vi "NV-ESR_Initialization.vi"() -> ()   [LabVIEW 2024]
panel:
  in  "Instructions":T1(array[cluster])=[{"Instruct Data"=0, "Op Code"=0, "Flags"=[FALSE, TRUE, TRUE, FALSE, FALSE, FALSE, FALSE, FALSE, FALSE, FALSE, FALSE, FALSE, FALSE, FALSE, FALSE, FALSE, FALSE, FALSE, FALSE, FALSE, FALSE, FALSE, FALSE, TRUE], "Comments"="0", "Time (s)"=1e-07}, {"Instruct Data"=0, "Op Code"=0, "Flags"=[TRUE, TRUE, FALSE, TRUE, FALSE, FALSE, FALSE, FALSE, FALSE, FALSE, FALSE, FALSE, FALSE, FALSE, FALSE, FALSE, FALSE, FALSE, FALSE, FALSE, FALSE, FALSE, FALSE, FALSE], "Comments"="1 MW", "Time (s)"=2e-06}, {"Instruct Data"=0, "Op Code"=6, "Flags"=[FALSE, TRUE, FALSE, FALSE, FALSE, FALSE, FALSE, FALSE, FALSE, FALSE, FALSE, FALSE, FALSE, FALSE, FALSE, FALSE, FALSE, FALSE, FALSE, FALSE, FALSE, FALSE, FALSE, FALSE], "Comments"="2 AOM delay", "Time (s)"=2e-06}, {"Instruct Data"=0, "Op Code"=0, "Flags"=[FALSE, TRUE, FALSE, FALSE, FALSE, FALSE, FALSE, FALSE, FALSE, FALSE, FALSE, FALSE, FALSE, FALSE, FALSE, FALSE, FALSE, FALSE, FALSE, FALSE, FALSE, FALSE, FALSE, FALSE], "Comments"="3 read", "Time (s)"=3e-07}, {"Instruct Data"=0, "Op Code"=0, "Flags"=[FALSE, TRUE, FALSE, FALSE, FALSE, FALSE, FALSE, TRUE, FALSE, FALSE, FALSE, FALSE, FALSE, FALSE, FALSE, FALSE, FALSE, FALSE, FALSE, FALSE, FALSE, FALSE, FALSE, FALSE], "Comments"="4 AOM", "Time (s)"=2.2e-06}, {"Instruct Data"=0, "Op Code"=6, "Flags"=[FALSE, FALSE, FALSE, FALSE, FALSE, FALSE, FALSE, TRUE, FALSE, FALSE, FALSE, FALSE, FALSE, FALSE, FALSE, FALSE, FALSE, FALSE, FALSE, FALSE, FALSE, FALSE, FALSE, FALSE], "Comments"="5", "Time (s)"=5e-06}, {"Instruct Data"=0, "Op Code"=6, "Flags"=[FALSE, TRUE, TRUE, FALSE, FALSE, FALSE, FALSE, FALSE, FALSE, FALSE, FALSE, FALSE, FALSE, FALSE, FALSE, FALSE, FALSE, FALSE, FALSE, FALSE, FALSE, FALSE, FALSE, FALSE], "Comments"="6", "Time (s)"=3e-06}, {"Instruct Data"=0, "Op Code"=0, "Flags"=[FALSE, TRUE, FALSE, FALSE, FALSE, FALSE, FALSE, FALSE, FALSE, FALSE, FALSE, FALSE, FALSE, FALSE, FALSE, FALSE, FALSE, FALSE, FALSE, FALSE, FALSE, FALSE, FALSE, FALSE], "Comments"="7", "Time (s)"=1e-06}, {"Instruct Data"=0, "Op Code"=0, "Flags"=[FALSE, TRUE, FALSE, FALSE, FALSE, FALSE, FALSE, FALSE, FALSE, FALSE, FALSE, FALSE, FALSE, FALSE, FALSE, FALSE, FALSE, FALSE, FALSE, FALSE, FALSE, FALSE, FALSE, FALSE], "Comments"="8", "Time (s)"=1e-06}, {"Instruct Data"=0, "Op Code"=0, "Flags"=[FALSE, TRUE, FALSE, FALSE, FALSE, FALSE, FALSE, FALSE, FALSE, FALSE, FALSE, FALSE, FALSE, FALSE, FALSE, FALSE, FALSE, FALSE, FALSE, FALSE, FALSE, FALSE, FALSE, FALSE], "Comments"="9", "Time (s)"=1e-06}] {"Time (s)" format="%.3p"; "Op Code" items=["Continue", "Stop", "Loop", "End Loop", "JSR", "RTS", "Branch", "Long Delay", "Wait"]}
  in  "Path to spinapi.dll":path=path "C:/SpinCore/SpinAPI/lib/spinapi64.dll"
  in  "# of Instructions":u32=3
  in  "clock_freq (MHz)":dbl=500.0
  # "1) MW indication\n2)AOM\n3) SR400 Trigger\n4)I\n5)Q\n24) Scope Trigger"
  # "1"
  # "2"
  # "3"
  # "4"
  # "5"
  # "6"
  # "7"
  # "8"
  # "9"
  # "10"
  # "11"
  # "12"
  # "13"
  # "14"
  # "15"
  # "16"
  # "17"
  # "18"
  # "19"
  # "20"
  # "21"
  # "22"
  # "23"
  # "24"
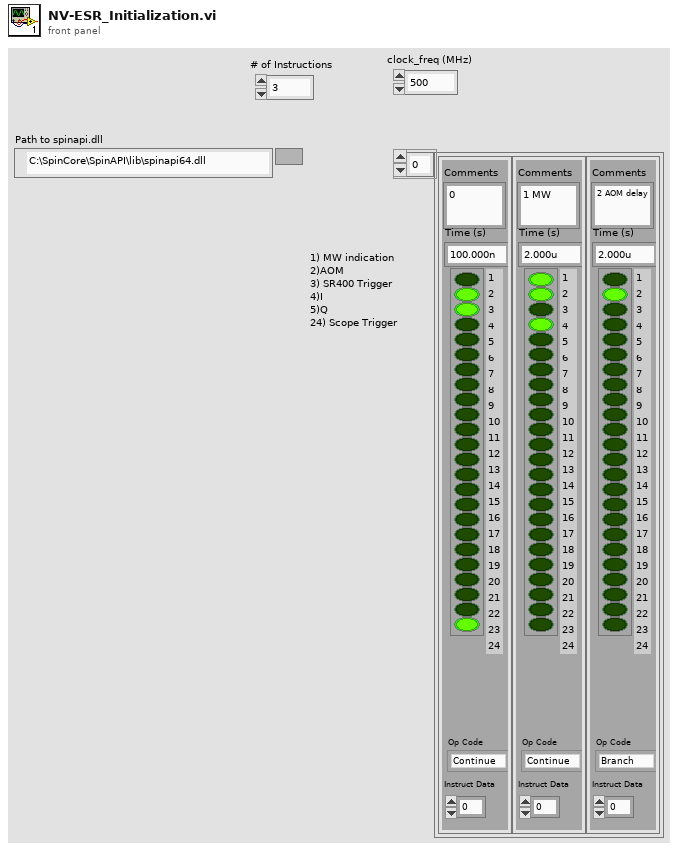
[diagram p1: front panel]
types:
  T1 = cluster{"Instruct Data":i32, "Op Code":i32, "Flags":bool[], "Comments":string, "Time (s)":dbl}[]
  T2 = enum16{"Pulse Program", "Frequency Registers", "TX Phase Registers", "RX Phase Registers"}
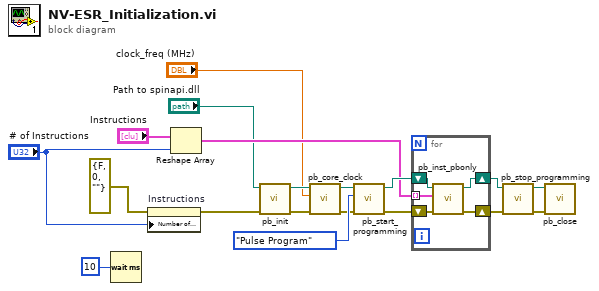
[diagram p0: block diagram]
diagram:
  n1 = Wait (ms)(milliseconds to wait=u32 10) -> ()  [unwired: 1 out]
  n2 = property on="Instructions" class="Arr (strict)"(error in=errorcluster {"status"=FALSE, "code"=0, "source"=""} ("error in (no error)"), "Number of Columns"="# of Instructions") -> (error out=w15:errorcluster)  [unwired: 1 in, 1 out]
  n3 = Reshape Array("Instructions", "# of Instructions") -> (w17:T1)
  n4 = call "pb_init.vi"("error in (no error)"=w15, "path in"="Path to spinapi.dll") -> ("error out"=w8:errorcluster, "path out"=w10:path)  [unwired: 2 in, 6 out]
  n5 = call "pb_core_clock.vi"("error in (no error)"=w8, "clock_freq (MHz)"="clock_freq (MHz)", "path in"=w10) -> ("error out"=w7:errorcluster, "path out"=w9:path)  [unwired: 7 in]
  n6 = call "pb_start_programming.vi"("error in (no error)"=w7, "Device"=T2."Pulse Program", "path in"=w9) -> ("error out"=w13:errorcluster, "path out"=w19:path)  [unwired: 1 in, 6 out]
  n7 = for {
    tunnel: w17 -> [w21] mode=indexing
    shift-right: [w23] -> w16
    shift-left: w19 -> [w24]
    shift-right: [w20] -> w12
    shift-left: w13 -> [w22]
    n8 = call "pb_inst_pbonly.vi"("error in (no error)"=w22, "PB Instruction"=w21, "path in"=w24) -> ("error out"=w20:errorcluster, "path out"=w23:path)  [unwired: 2 in, 5 out]
  }
  n9 = call "pb_stop_programming.vi"("error in (no error)"=w12, "path in"=w16) -> ("error out"=w11:errorcluster, "path out"=w18:path)  [unwired: 1 in, 7 out]
  n10 = call "pb_close.vi"("error in (no error)"=w11, "path in"=w18) -> ()  [unwired: 10 out]
